vi "VM Spy - format history info for variable list.vi"(9 "Has history":bool, 10 "Variable name":string, 11 "VC Handle":T1=-1) -> (3 "String out":string)   [LabVIEW 2021]
doc: "::: CalcExpress Toolkit :::\nCopyright (c) 2000-2026 Konstantin Shifershteyn. All rights reserved."
uses:
  vi.lib/addons/CalcExpress/cetypes.llb/VarMan Variable Context Handle.ctl
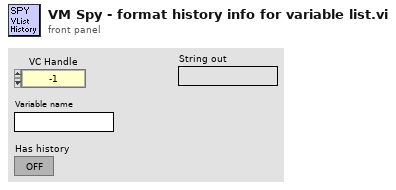
[diagram p1: front panel]
types:
  T1 = typedef "VarMan Variable Context Handle.ctl" = i32
  T2 = enum32{"nop", "create", "destroy", "reset", "get info", "config", "create_wrid"}
  T3 = typedef "VarMan History Info.ctl" = cluster{"var type":u32, "history length":u32, "stored values":u32, "update cnt":u32, "last update ms":u32, "newest timestamp":dbl, "oldest timestamp":dbl, "NewVals mode":cluster{"NewVals cnt":u32, "last read time":dbl, "last read ms":u32}, "time condition":cluster{"Step, ms":u32, "Gate, ms":u32}, "value condition":cluster{"condition":enum32{"don't test", "changed", "abs deviation", "rel deviation", "out of range", "within range"}, "Delta":dbl, "Range_Min":dbl, "Range_Max":dbl}}
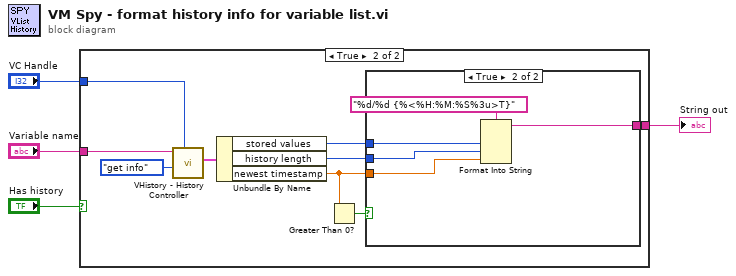
[diagram p0: block diagram]
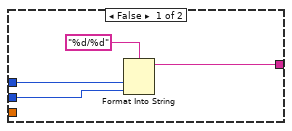
[diagram p3: hidden frame]
diagram:
  n1 = case shown="True" "Has history" {
    tunnel: "Variable name" -> [_ w13]
    tunnel: "VC Handle" -> [_ w12]
    tunnel: [_ w9] -> w1
    frame False {
    }
    frame True {
      n2 = call "VHistory - History Controller.vi"("VC Handle"=w12, "cmd (nop:default)"=T2."get info", "name_spec"=w13) -> ("history info"=w11:T3)  [unwired: 5 in, 3 out]
      n3 = Unbundle By Name(w11) -> ("stored values"=w10:u32, "history length"=w6:u32, "newest timestamp"=w7:dbl)
      n4 = Greater Than 0?(x=w7) -> (x > 0?=w8:bool)
      n5 = case shown="True" w8 {
        tunnel: w7 -> [_ w21]
        tunnel: w10 -> [w16 w20]
        tunnel: [w15 w19] -> w9
        tunnel: w6 -> [w14 w18]
        frame False {
          n6 = Format Into String(format string="%d/%d", w16, w14) -> (resulting string=w15:string)  [unwired: 2 in, 1 out]
        }
        frame True {
          n7 = Format Into String(format string="%d/%d {%<%H:%M:%S%3u>T}", w20, w18, w21) -> (resulting string=w19:string)  [unwired: 2 in, 1 out]
        }
      }
    }
  }
  "String out" <- w1
